vi "VI Reference Includes.vi"   [LabVIEW 2014, in "Engine Runtime Interface.lvclass"]
uses:
  Engine Runtime Interface.lvclass
  Engine Configuration/add and map fixed channel mapping.vi
  Engine Configuration/rename channel in mapping.vi
  Engine Configuration/apply mapping changes.vi
  Engine Configuration/delete mapping by channel.vi
  Engine Configuration/add mapping.vi
  Engine Configuration/apply tag changes.vi
  Engine Configuration/locate tag by name.vi
  Engine Configuration/delete tag.vi
  Engine Configuration/change tag metadata.vi
  Engine Configuration/change tag raw default value.vi
  Engine Configuration/change tag type.vi
  Engine Configuration/rename tag.vi
  Engine Configuration/add tag.vi
  Engine Configuration/Mappings.ctl
  Engine Configuration/Module Mappings.ctl
  Engine Configuration/Tag Info.ctl
  Engine Configuration/filter tags by writer.vi
  Engine Configuration/filter tags by owner.vi
  Engine Configuration/filter tags by readers.vi
  Engine Configuration/filter tags available for mapping to channel.vi
  Engine Configuration/get full tag list.vi
  Engine Configuration/find tag mapped to channel.vi
  Engine Configuration/from string.vi
  Engine Configuration/to string.vi
  Execution States.ctl
  Open.vi
  Initialize.vi
  Start.vi
  Set Safe State.vi
  Pause.vi
  Get State.vi
  Stop.vi
  Close.vi
  Discover Channels.vi
  Engine Configuration/dynamic tag creation and mapping.vi
  Engine Configuration/delete module from engine.vi
  Engine Configuration/is module registered.vi
  Engine Configuration/add module to engine.vi
  Engine Configuration/engine configuration.lvclass
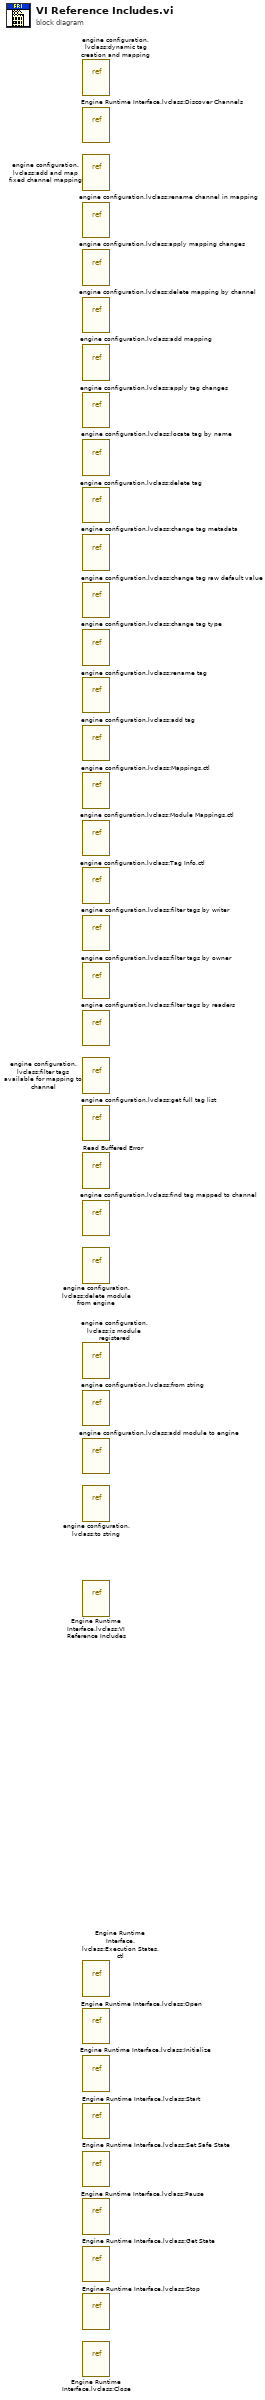
[diagram p0: block diagram]
diagram:
  n1 = vi-ref "engine configuration.lvclass:dynamic tag creation and mapping.vi"() -> ()  [unwired: 1 out]
  n2 = vi-ref "Engine Runtime Interface.lvclass:Discover Channels.vi"() -> ()  [unwired: 1 out]
  n3 = vi-ref "engine configuration.lvclass:add and map fixed channel mapping.vi"() -> ()  [unwired: 1 out]
  n4 = vi-ref "engine configuration.lvclass:rename channel in mapping.vi"() -> ()  [unwired: 1 out]
  n5 = vi-ref "engine configuration.lvclass:apply mapping changes.vi"() -> ()  [unwired: 1 out]
  n6 = vi-ref "engine configuration.lvclass:delete mapping by channel.vi"() -> ()  [unwired: 1 out]
  n7 = vi-ref "engine configuration.lvclass:add mapping.vi"() -> ()  [unwired: 1 out]
  n8 = vi-ref "engine configuration.lvclass:apply tag changes.vi"() -> ()  [unwired: 1 out]
  n9 = vi-ref "engine configuration.lvclass:locate tag by name.vi"() -> ()  [unwired: 1 out]
  n10 = vi-ref "engine configuration.lvclass:delete tag.vi"() -> ()  [unwired: 1 out]
  n11 = vi-ref "engine configuration.lvclass:change tag metadata.vi"() -> ()  [unwired: 1 out]
  n12 = vi-ref "engine configuration.lvclass:change tag raw default value.vi"() -> ()  [unwired: 1 out]
  n13 = vi-ref "engine configuration.lvclass:change tag type.vi"() -> ()  [unwired: 1 out]
  n14 = vi-ref "engine configuration.lvclass:rename tag.vi"() -> ()  [unwired: 1 out]
  n15 = vi-ref "engine configuration.lvclass:add tag.vi"() -> ()  [unwired: 1 out]
  n16 = vi-ref "engine configuration.lvclass:Mappings.ctl"() -> ()  [unwired: 1 out]
  n17 = vi-ref "engine configuration.lvclass:Module Mappings.ctl"() -> ()  [unwired: 1 out]
  n18 = vi-ref "engine configuration.lvclass:Tag Info.ctl"() -> ()  [unwired: 1 out]
  n19 = vi-ref "engine configuration.lvclass:filter tags by writer.vi"() -> ()  [unwired: 1 out]
  n20 = vi-ref "engine configuration.lvclass:filter tags by owner.vi"() -> ()  [unwired: 1 out]
  n21 = vi-ref "engine configuration.lvclass:filter tags by readers.vi"() -> ()  [unwired: 1 out]
  n22 = vi-ref "engine configuration.lvclass:filter tags available for mapping to channel.vi"() -> ()  [unwired: 1 out]
  n23 = vi-ref "engine configuration.lvclass:get full tag list.vi"() -> ()  [unwired: 1 out]
  n24 = vi-ref "Read Buffered Error.vi"() -> ()  [unwired: 1 out]
  n25 = vi-ref "engine configuration.lvclass:find tag mapped to channel.vi"() -> ()  [unwired: 1 out]
  n26 = vi-ref "engine configuration.lvclass:delete module from engine.vi"() -> ()  [unwired: 1 out]
  n27 = vi-ref "engine configuration.lvclass:is module registered.vi"() -> ()  [unwired: 1 out]
  n28 = vi-ref "engine configuration.lvclass:from string.vi"() -> ()  [unwired: 1 out]
  n29 = vi-ref "engine configuration.lvclass:add module to engine.vi"() -> ()  [unwired: 1 out]
  n30 = vi-ref "engine configuration.lvclass:to string.vi"() -> ()  [unwired: 1 out]
  n31 = vi-ref "Engine Runtime Interface.lvclass:VI Reference Includes.vi"() -> ()  [unwired: 1 out]
  n32 = vi-ref "Engine Runtime Interface.lvclass:Execution States.ctl"() -> ()  [unwired: 1 out]
  n33 = vi-ref "Engine Runtime Interface.lvclass:Open.vi"() -> ()  [unwired: 1 out]
  n34 = vi-ref "Engine Runtime Interface.lvclass:Initialize.vi"() -> ()  [unwired: 1 out]
  n35 = vi-ref "Engine Runtime Interface.lvclass:Start.vi"() -> ()  [unwired: 1 out]
  n36 = vi-ref "Engine Runtime Interface.lvclass:Set Safe State.vi"() -> ()  [unwired: 1 out]
  n37 = vi-ref "Engine Runtime Interface.lvclass:Pause.vi"() -> ()  [unwired: 1 out]
  n38 = vi-ref "Engine Runtime Interface.lvclass:Get State.vi"() -> ()  [unwired: 1 out]
  n39 = vi-ref "Engine Runtime Interface.lvclass:Stop.vi"() -> ()  [unwired: 1 out]
  n40 = vi-ref "Engine Runtime Interface.lvclass:Close.vi"() -> ()  [unwired: 1 out]
